vi "Configure Session.vi"(8 "error in":errorcluster, 11 "Plugin in":refnum<class "DFT_Spectra.lvclass">) -> (0 "error out":errorcluster, 3 "Plugin out":refnum<class "DFT_Spectra.lvclass">)   [LabVIEW 2024, in "DFT_Spectra.lvlib" / "DFT_Spectra.lvclass"]
uses:
  DFT_Spectra.lvclass
  DFT_Spectra Data.ctl
  <vilib>/Analysis/4window.llb/windowTd.ctl
  <vilib>/addons/_NISVFA/_Shared subVIs/Data Objects/Waveforms (DBL)/Waveforms (N Ch).lvclass
  <vilib>/FlexLogger/SDK/PluginSDK.lvlibp/PEFClasses/SDK/Processing Element/Timing Parameters.ctl
  <vilib>/FlexLogger/SDK/PluginSDK.lvlibp/PEFClasses/SDK/Processing Element/Timing Method.ctl
  <vilib>/FlexLogger/SDK/PluginSDK.lvlibp/PEFClasses/SDK/System Interface/Resampling Mode.ctl
  DFT_Spectra.lvclass/DFT_Spectra.ctl
  DFT_Spectra Global.vi
  <vilib>/FlexLogger/SDK/PluginSDK.lvlibp/PEFClasses/SDK/Plugin/ParameterAccess/Read DBL.vi
  <vilib>/FlexLogger/SDK/PluginSDK.lvlibp/PEFClasses/SDK/Plugin/ParameterAccess/Read Enum.vi
  <vilib>/FlexLogger/SDK/PluginSDK.lvlibp/PEFClasses/SDK/Plugin/ParameterAccess/Read I32.vi
  <vilib>/addons/_NISVFA/_Shared subVIs/Data Objects/Data/Data.lvclass
  <vilib>/FlexLogger/SDK/PluginSDK.lvlibp/PEFClasses/SDK/Plugin/Plugin.lvclass
  <vilib>/Utility/LVLibp/NI_PackedLibraryUtility.lvlib
  <vilib>/Analysis/NI_AALPro.lvlib
  <vilib>/FlexLogger/SDK/PluginSDK.lvlibp/PEFClasses/SDK/Processing Element/Processing Element.lvclass
  <vilib>/FlexLogger/SDK/PluginSDK.lvlibp/PEFClasses/SDK/System Interface/System Interface.lvclass
  C:/Program Files/National Instruments/LabVIEW 2024/vi.lib/FlexLogger/SDK/PluginSDK.lvlibp/PEFClasses/SDK/Plugin/Plugin.lvclass
  C:/Program Files/National Instruments/LabVIEW 2024/vi.lib/FlexLogger/SDK/PluginSDK.lvlibp/PEFClasses/SDK/Processing Element/Processing Element.lvclass
  C:/dev/dsb/niflexlogger-plugins/PDK plugins/DFT_Spectra/source/DFT_Spectra.lvclass
  <vilib>/FlexLogger/SDK/PluginSDK.lvlibp/PEFClasses/SDK/Plugin/ParameterAccess/Write I32.vi
  <vilib>/FlexLogger/SDK/PluginSDK.lvlibp/PEFClasses/SDK/Plugin/ParameterAccess/Write DBL.vi
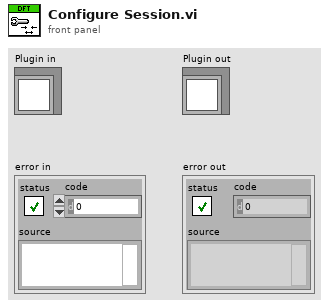
[diagram p1: front panel]
types:
  T1 = cluster{"averaging mode":enum16{"No averaging", "Vector averaging", "RMS averaging", "Peak hold"}, "weighting mode":enum16{"Linear", "Exponential"}, "number of averages":u32}
  T2 = typedef "PluginSDK.lvlibp/System Interface.lvclass/Resampling Mode.ctl" = enum16{"No Resampling", "Custom Rate", "Maximum Rate", "Minimum Rate"}
  T3 = typedef "PluginSDK.lvlibp/Processing Element.lvclass/Timing Parameters.ctl" = cluster{"Timing Method":T4, "Timing Period (ms)":i32}
  T4 = typedef "PluginSDK.lvlibp/Processing Element.lvclass/Timing Method.ctl" = enum16{"Periodic", "Immediate", "On Data Ready", "Triggered"}
  T5 = typedef "DFT_Spectra.lvlib/DFT_Spectra.lvclass/DFT_Spectra Data.ctl" = cluster{"First Time":bool, "Show Results Window":bool, "Show Results Window Clicked":bool, "Window":T6, "overlap":i32, "Block Duration":dbl, "Averaging parameters":cluster{"averaging mode":enum16{"No averaging", "Vector averaging", "RMS averaging", "Peak hold"}, "weighting mode":enum16{"Linear", "Exponential"}, "number of averages":u32}, "buffer out":refnum<data-value>, "Avg Spectra":refnum<vi>, "Spectra UI":refnum<vi>}
  T6 = typedef "NI_AALPro.lvlib/windowTd.ctl" = u32
  T7 = enum16{"No averaging", "Vector averaging", "RMS averaging", "Peak hold"}[]
  T8 = enum16{"No averaging", "Vector averaging", "RMS averaging", "Peak hold"}
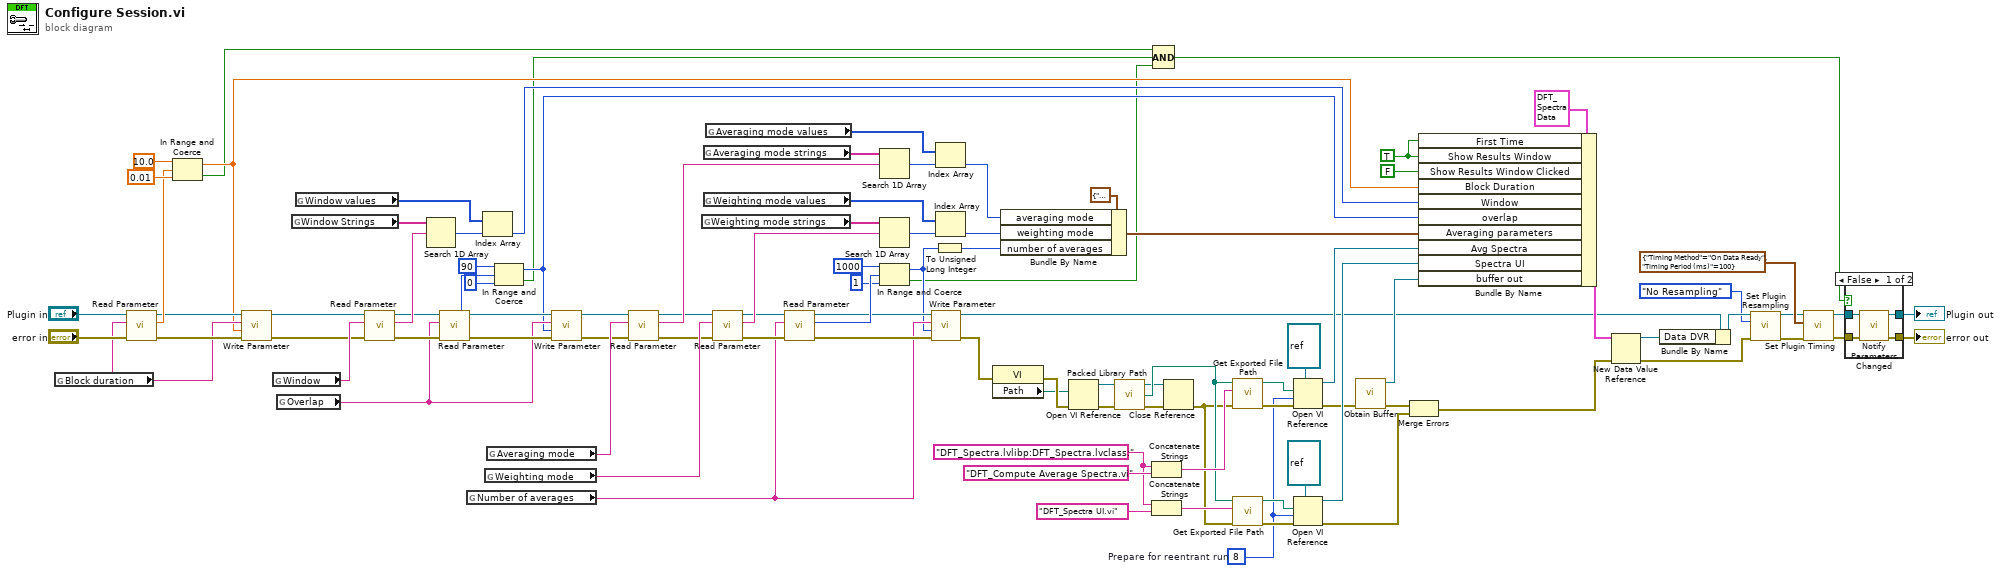
[diagram p0: block diagram]
diagram:
  w43 = "DFT_Spectra.lvlibp:DFT_Spectra.lvclass:" ("qualified name")
  w46 = 8  # Prepare for reentrant run
  w101 = TRUE ("Show Spectrogram Window")
  n1 = global read "DFT_Spectra Global.vi" "Block duration"() -> (w22:string)
  n2 = call-poly <vilib>:"Read Parameter.vi"("error in (no error)"="error in", "Name"=w22, "Plugin in"="Plugin in") -> ("error out"=w25:errorcluster, "Value"=w28:dbl, "Plugin out"=w26:refnum<class "DFT_Spectra.lvclass">)  [unwired: 5 in, 1 out]
  n3 = In Range and Coerce(upper limit=10.0, x=w28, lower limit=0.01) -> (coerced(x)=w21:dbl, In Range?=w8:bool)
  n4 = call-poly <vilib>:"Write Parameter.vi"("error in (no error)"=w25, "Value"=w21, "Name"=w22, "Plugin in"=w26) -> ("error out"=w23:errorcluster, "Plugin out"=w24:refnum<class "DFT_Spectra.lvclass">)  [unwired: 6 in]
  n5 = global read "DFT_Spectra Global.vi" "Window"() -> (w95:string)
  n6 = global read "DFT_Spectra Global.vi" "Overlap"() -> (w16:string)
  n7 = global read "DFT_Spectra Global.vi" "Window Strings"() -> (w96:string[])
  n8 = global read "DFT_Spectra Global.vi" "Window values"() -> (w97:u32[])
  n9 = call-poly <vilib>:"Read Parameter.vi"("error in (no error)"=w23, "Name"=w95, "Plugin in"=w24) -> ("error out"=w68:errorcluster, "Value"=w99:string, "Plugin out"=w69:refnum<class "DFT_Spectra.lvclass">)  [unwired: 4 in, 2 out]
  n10 = Search 1D Array(1D array=w96, element=w99) -> (index of element=w98:i32)  [unwired: 1 in]
  n11 = call-poly <vilib>:"Read Parameter.vi"("error in (no error)"=w68, "Name"=w16, "Plugin in"=w69) -> ("error out"=w19:errorcluster, "Value"=w31:i32, "Plugin out"=w20:refnum<class "DFT_Spectra.lvclass">)  [unwired: 5 in, 1 out]
  n12 = global read "DFT_Spectra Global.vi" "Number of averages"() -> (w10:string)
  n13 = Index Array(array=w97, index=w98) -> (element=w27:u32)
  n14 = global read "DFT_Spectra Global.vi" "Weighting mode"() -> (w85:string)
  n15 = global read "DFT_Spectra Global.vi" "Averaging mode"() -> (w90:string)
  n16 = In Range and Coerce(upper limit=90, x=w31, lower limit=0) -> (coerced(x)=w15:i32, In Range?=w7:bool)
  n17 = call-poly <vilib>:"Write Parameter.vi"("error in (no error)"=w19, "Value"=w15, "Name"=w16, "Plugin in"=w20) -> ("error out"=w17:errorcluster, "Plugin out"=w18:refnum<class "DFT_Spectra.lvclass">)  [unwired: 6 in]
  n18 = call-poly <vilib>:"Read Parameter.vi"("error in (no error)"=w17, "Name"=w90, "Plugin in"=w18) -> ("error out"=w83:errorcluster, "Value"=w94:string, "Plugin out"=w84:refnum<class "DFT_Spectra.lvclass">)  [unwired: 4 in, 2 out]
  n19 = global read "DFT_Spectra Global.vi" "Weighting mode strings"() -> (w86:string[])
  n20 = global read "DFT_Spectra Global.vi" "Averaging mode strings"() -> (w91:string[])
  n21 = global read "DFT_Spectra Global.vi" "Weighting mode values"() -> (w87:enum16{"Linear", "Exponential"}[])
  n22 = global read "DFT_Spectra Global.vi" "Averaging mode values"() -> (w92:T7)
  n23 = call-poly <vilib>:"Read Parameter.vi"("error in (no error)"=w83, "Name"=w85, "Plugin in"=w84) -> ("error out"=w81:errorcluster, "Value"=w89:string, "Plugin out"=w82:refnum<class "DFT_Spectra.lvclass">)  [unwired: 4 in, 2 out]
  n24 = call-poly <vilib>:"Read Parameter.vi"("error in (no error)"=w81, "Name"=w10, "Plugin in"=w82) -> ("error out"=w12:errorcluster, "Value"=w64:i32, "Plugin out"=w14:refnum<class "DFT_Spectra.lvclass">)  [unwired: 5 in, 1 out]
  n25 = Search 1D Array(1D array=w91, element=w94) -> (index of element=w93:i32)  [unwired: 1 in]
  n26 = Search 1D Array(1D array=w86, element=w89) -> (index of element=w88:i32)  [unwired: 1 in]
  n27 = In Range and Coerce(upper limit=1000, x=w64, lower limit=1) -> (coerced(x)=w9:i32, In Range?=w6:bool)
  n28 = call-poly <vilib>:"Write Parameter.vi"("error in (no error)"=w12, "Value"=w9, "Name"=w10, "Plugin in"=w14) -> ("error out"=w11:errorcluster, "Plugin out"=w13:refnum<class "DFT_Spectra.lvclass">)  [unwired: 6 in]
  n29 = To Unsigned Long Integer(number=w9) -> (unsigned 32bit integer=w77:u32)
  n30 = Index Array(array=w92, index=w93) -> (element=w79:T8)
  n31 = Index Array(array=w87, index=w88) -> (element=w78:enum16{"Linear", "Exponential"})
  n32 = property class="VI"(error in=w11) -> (error out=w53:errorcluster, "Path"=w40:path)  [unwired: 1 in, 1 out]
  n33 = Bundle By Name(cluster=T1 {"averaging mode"=enum."No averaging", "weighting mode"=enum."Linear", "number of averages"=0} ("Averaging parameters"), "averaging mode"=w79, "weighting mode"=w78, "number of averages"=w77) -> (w50:T1)
  n34 = Open VI Reference(vi path=w40, error in (no error)=w53) -> (vi reference=w51:refnum<vi>, error out=w52:errorcluster)  [unwired: 4 in]
  n35 = call <vilib>:"Packed Library Path.vi"("error in (no error)"=w52, "vi reference"=w51) -> ("error out"=w38:errorcluster, "packed library path"=w39:path, "vi reference out"=w36:refnum<vi>)  [unwired: 1 in]
  n36 = Concatenate Strings(w43, "DFT_Compute Average Spectra.vi" ("qualified name")) -> (w44:string)
  n37 = Concatenate Strings(w43, "DFT_Spectra UI.vi" ("qualified name")) -> (w41:string)
  n38 = Compound Arithmetic op=AND(w8, w7, w6) -> (w5:bool)
  n39 = Close Reference(reference=w36, error in (no error)=w38) -> (error out=w37:errorcluster)
  n40 = call <vilib>:"Get Exported File Path.vi"("error in (no error)"=w37, "qualified name"=w44, "packed library path"=w39) -> ("error out"=w56:errorcluster, "path"=w55:path)  [unwired: 7 in]
  n41 = call <vilib>:"Get Exported File Path.vi"("error in (no error)"=w37, "qualified name"=w41, "packed library path"=w39) -> ("error out"=w58:errorcluster, "path"=w59:path)  [unwired: 7 in]
  n42 = Open VI Reference(type specifier VI Refnum (for type only)=refnum<vi> refnum, vi path=w55, options=w46, error in (no error)=w56) -> (vi reference=w47:refnum<vi>, error out=w49:errorcluster)  [unwired: 2 in]
  n43 = Open VI Reference(type specifier VI Refnum (for type only)=refnum<vi> refnum, vi path=w59, options=w46, error in (no error)=w58) -> (vi reference=w72:refnum<vi>, error out=w67:errorcluster)  [unwired: 2 in]
  n44 = call <vilib>:"Obtain Buffer.vi"("error in (no error)"=w49) -> ("error out"=w48:errorcluster, "buffer out"=w57:refnum<data-value>)  [unwired: 9 in]
  n45 = Merge Errors(w48, w67) -> (w35:errorcluster)
  n46 = Bundle By Name(cluster=T5 {"First Time"=FALSE, "Show Results Window"=FALSE, "Show Results Window Clicked"=FALSE, "Window"=0, "overlap"=0, "Block Duration"=0.0, "Averaging parameters"={"averaging mode"=enum."No averaging", "weighting mode"=enum."Linear", "number of averages"=0}, "buffer out"=refnum, "Avg Spectra"=refnum, "Spectra UI"=refnum} ("Data"), "First Time"=w101, "Show Results Window"=w101, "Show Results Window Clicked"=FALSE ("Show Spectrogram Window"), "Block Duration"=w21, "Window"=w27, "overlap"=w15, "Averaging parameters"=w50, "Avg Spectra"=w47, "Spectra UI"=w72, "buffer out"=w57) -> (w61:T5)
  n47 = New Data Value Reference(data value=w61, error in=w35) -> (data value reference=w76:refnum<data-value>, error out=w34:errorcluster)
  n48 = Bundle By Name(cluster=w13, "Data DVR"=w76) -> (w74:refnum<class "DFT_Spectra.lvclass">)
  n49 = call <vilib>:"Set Plugin Resampling.vi"("Plugin in"=w74, "Resampling Mode"=Resampling_Mode."No Resampling", "error in (no error)"=w34) -> ("Plugin out"=w66:refnum<class "DFT_Spectra.lvclass">, "error out"=w65:errorcluster)  [unwired: 11 in]
  n50 = call <vilib>:"Set Plugin Timing.vi"("error in (no error)"=w65, "Timing Parameters"=T3 {"Timing Method"=enum."On Data Ready", "Timing Period (ms)"=100}, "Plugin in"=w66) -> ("error out"=w4:errorcluster, "Plugin out"=w3:refnum<class "DFT_Spectra.lvclass">)  [unwired: 7 in]
  n51 = case shown="False" w5 {
    tunnel: w4 -> [w106 w107]
    tunnel: w3 -> [w105 w108]
    tunnel: [w104 w108] -> w2
    tunnel: [w103 w107] -> w1
    frame False {
      n52 = call <vilib>:"Notify Parameters Changed.vi"("error in (no error)"=w106, "Plugin in"=w105) -> ("error out"=w103:errorcluster, "Plugin out"=w104:refnum<class "DFT_Spectra.lvclass">)  [unwired: 8 in]
    }
    frame True {
    }
  }
  "error out" <- w1
  "Plugin out" <- w2
